vi "Test Project Edits.vi"(8 "error in":errorcluster, 10 "Work Folder":path, 11 "Test Data Folder":path) -> (0 "error out":errorcluster, 2 "Report":string, 3 "Passed":bool)   [LabVIEW 2026]
doc: "Tests Set Task Active.vi and Save Project.vi on a copy of the schema-v2 sample data. Every check reads the data back from disk with a fresh Initialize Stores.vi. Checks: Meetings set inactive is left out of the TimeTracker task list after re-reading; a new project with two tasks survives re-reading; saving it again with one extra name adds only that task and keeps the IDs of the others; an unknown Project ID returns error 5102.\n\nInputs: Test Data Folder; Work Folder; error in. Outputs: Passed; Report; error out.\n\nGenerated by: Claude"
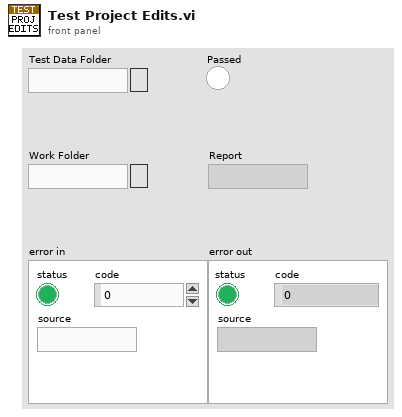
[diagram p1: front panel]
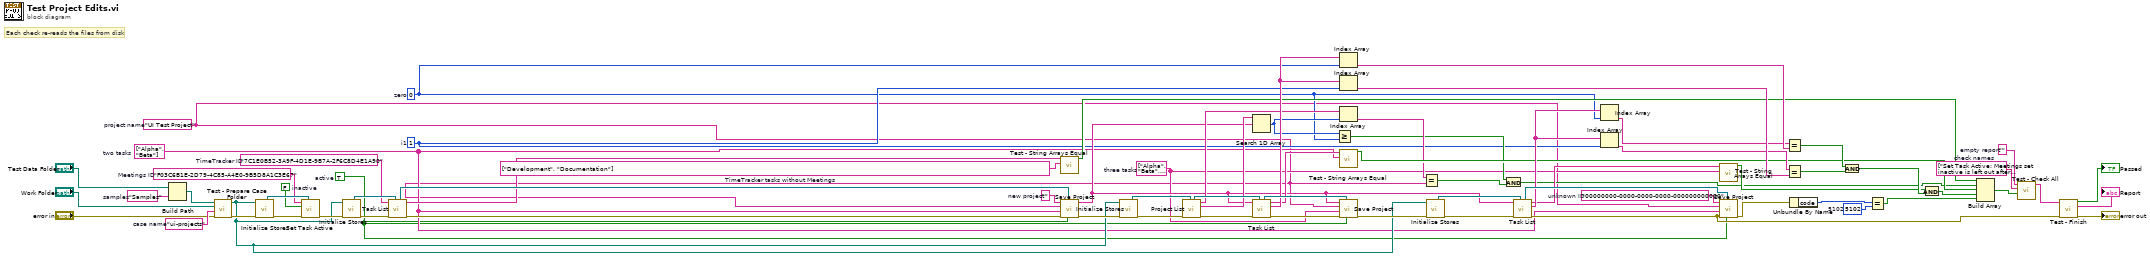
[diagram p0: block diagram]
diagram:
  w23 = string[] ["Set Task Active: Meetings set inactive is left out after re-reading", "Save Project: new project gets an ID and is listed after re-reading", "Save Project: its two tasks survive re-reading", "Save Project: saving again adds only the new task and keeps the other IDs", "Save Project: unknown Project ID gives error 5102"]  # check names
  w22 = string[] ["Development", "Documentation"]  # TimeTracker tasks without Meetings
  w21 = 1  # i1
  w20 = 0  # zero
  w19 = 5102  # 5102
  w18 = "00000000-0000-0000-0000-000000000000"  # unknown ID
  w17 = string[] ["Alpha", "Beta", "Gamma"]  # three tasks
  w16 = string[] ["Alpha", "Beta"]  # two tasks
  w15 = "UI Test Project"  # project name
  w14 = ""  # new project
  w13 = TRUE  # active
  w12 = FALSE  # inactive
  w11 = "F03C6B1E-2D79-4C85-A4E0-9B5D8A1C3E67"  # Meetings ID
  w10 = "7C1E0B52-3A9F-4D1E-9B7A-2F6C8D4E1A90"  # TimeTracker ID
  w9 = ""  # empty report
  w8 = "ui-projects"  # case name
  w7 = "Samples"  # samples
  # "Each check re-reads the files from disk"
  n1 = Build Path(base path="Test Data Folder", name or relative path=w7) -> (appended path=w24:path)
  n2 = call "Test - Prepare Case Folder.vi"("error in (no error)"="error in", "Case Name"=w8, "Work Folder"="Work Folder", "Source Folder"=w24) -> ("error out"=w26:errorcluster, "Case Folder"=w25:path)  [unwired: 6 in]
  n3 = call "Initialize Stores.vi"("error in"=w26, "Data Folder"=w25) -> ("error out"=w28:errorcluster, "Project Store out"=w27:refnum<class "Project Store.lvclass">)  [unwired: 5 in, 3 out]
  n4 = call "Set Task Active.vi"("Project Store in"=w27, "error in"=w28, "Active?"=w12, "Task ID"=w11) -> ("error out"=w29:errorcluster)  [unwired: 6 in, 1 out]
  n5 = call "Initialize Stores.vi"("error in"=w29, "Data Folder"=w25) -> ("error out"=w31:errorcluster, "Project Store out"=w30:refnum<class "Project Store.lvclass">)  [unwired: 5 in, 3 out]
  n6 = call "Task List.vi"("Project Store in"=w30, "error in"=w31, "Project ID"=w10) -> ("error out"=w34:errorcluster, "Task Names"=w32:string[], "Project Store out"=w33:refnum<class "Project Store.lvclass">)  [unwired: 5 in, 1 out]
  n7 = call "Test - String Arrays Equal.vi"("Expected"=w22, "Actual"=w32) -> ("Equal?"=w35:bool)  [unwired: 8 in, 1 out]
  n8 = call "Save Project.vi"("Project Active?"=w13, "Project Store in"=w33, "error in"=w34, "Task Names"=w16, "Project Name"=w15, "Project ID"=w14) -> ("error out"=w37:errorcluster, "Project ID out"=w36:string)  [unwired: 3 in, 1 out]
  n9 = call "Initialize Stores.vi"("error in"=w37, "Data Folder"=w25) -> ("error out"=w39:errorcluster, "Project Store out"=w38:refnum<class "Project Store.lvclass">)  [unwired: 5 in, 3 out]
  n10 = call "Project List.vi"("Project Store in"=w38, "error in"=w39) -> ("error out"=w43:errorcluster, "Project IDs"=w41:string[], "Project Names"=w40:string[], "Project Store out"=w42:refnum<class "Project Store.lvclass">)  [unwired: 6 in]
  n11 = Search 1D Array(1D array=w41, element=w36) -> (index of element=w44:i32)  [unwired: 1 in]
  n12 = call "Task List.vi"("Project Store in"=w42, "error in"=w43, "Project ID"=w36) -> ("error out"=w52:errorcluster, "Task IDs"=w50:string[], "Task Names"=w49:string[], "Project Store out"=w51:refnum<class "Project Store.lvclass">)  [unwired: 5 in]
  n13 = Greater Or Equal?(x=w44, y=w20) -> (x >= y?=w45:bool)
  n14 = Index Array(array=w50, index=w20) -> (element=w64:string)
  n15 = Index Array(array=w50, index=w21) -> (element=w65:string)
  n16 = Index Array(array=w40, index=w44) -> (element=w46:string)
  n17 = call "Test - String Arrays Equal.vi"("Expected"=w16, "Actual"=w49) -> ("Equal?"=w53:bool)  [unwired: 8 in, 1 out]
  n18 = call "Save Project.vi"("Project Active?"=w13, "Project Store in"=w51, "error in"=w52, "Task Names"=w17, "Project Name"=w15, "Project ID"=w36) -> ("error out"=w54:errorcluster)  [unwired: 3 in, 2 out]
  n19 = Equal?(x=w46, y=w15) -> (x = y?=w47:bool)
  n20 = call "Initialize Stores.vi"("error in"=w54, "Data Folder"=w25) -> ("error out"=w56:errorcluster, "Project Store out"=w55:refnum<class "Project Store.lvclass">)  [unwired: 5 in, 3 out]
  n21 = And(x=w45, y=w47) -> (x .and. y?=w48:bool)
  n22 = call "Task List.vi"("Project Store in"=w55, "error in"=w56, "Project ID"=w36) -> ("error out"=w60:errorcluster, "Task IDs"=w58:string[], "Task Names"=w57:string[], "Project Store out"=w59:refnum<class "Project Store.lvclass">)  [unwired: 5 in]
  n23 = Index Array(array=w58, index=w20) -> (element=w62:string)
  n24 = Index Array(array=w58, index=w21) -> (element=w63:string)
  n25 = call "Test - String Arrays Equal.vi"("Expected"=w17, "Actual"=w57) -> ("Equal?"=w61:bool)  [unwired: 8 in, 1 out]
  n26 = call "Save Project.vi"("Project Active?"=w13, "Project Store in"=w59, "error in"=w60, "Task Names"=w16, "Project Name"=w15, "Project ID"=w18) -> ("error out"=w70:errorcluster)  [unwired: 3 in, 2 out]
  n27 = Equal?(x=w62, y=w64) -> (x = y?=w66:bool)
  n28 = Equal?(x=w63, y=w65) -> (x = y?=w67:bool)
  n29 = Unbundle By Name(w70) -> ("code"=w71:i32)
  n30 = And(x=w66, y=w67) -> (x .and. y?=w68:bool)
  n31 = Equal?(x=w71, y=w19) -> (x = y?=w72:bool)
  n32 = And(x=w61, y=w68) -> (x .and. y?=w69:bool)
  n33 = Build Array(w35, w48, w53, w69, w72) -> (w73:bool[])
  n34 = call "Test - Check All.vi"("Conditions"=w73, "Check Names"=w23, "Report in"=w9) -> ("Report out"=w74:string)  [unwired: 7 in, 1 out]
  n35 = call "Test - Finish.vi"("error in (no error)"=w60, "Report"=w74) -> ("error out"=→"error out":errorcluster, "Report out"=→"Report":string, "Passed"=→"Passed":bool)  [unwired: 7 in]
